vi "_CalcExpress Examples Navigator.vi"   [LabVIEW 2021]
doc: "This VI launches <B>CalcExpress Examples Navigator</B> which will help you to explore CalcExpress examples.\n\nYou can also start the Examples Navigator through <B>Tools>>CalcExpress</B> menu.\n\n::: CalcExpress Toolkit :::\nCopyright (c) 2000-2026 Konstantin Shifershteyn. All rights reserved."
uses:
  vi.lib/addons/CalcExpress/cemisc.llb/[ce] CE component paths - Kind of Path Enum.ctl
panel:
  # "Starting CalcExpress Examples Navigator..."
types:
  T1 = typedef "[ce] CE component paths - Kind of Path Enum.ctl" = enum16{"VIs", "FuncVIs", "Help", "Examples", "Project", "Templates"}
  T2 = enum32{"Invalid", "Standard", "Closed", "Hidden", "Minimized", "Maximized"}
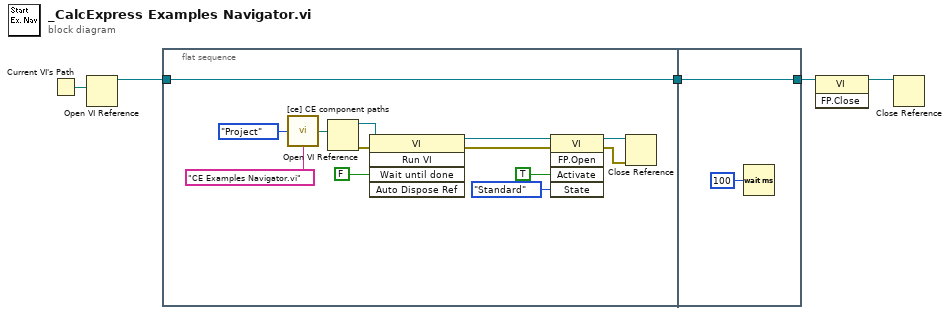
[diagram p0: block diagram]
diagram:
  n1 = Current VI's Path() -> (path=w5:path)
  n2 = Open VI Reference(vi path=w5) -> (vi reference=w2:refnum<vi>)  [unwired: 5 in, 1 out]
  n3 = flat-sequence {
    tunnel: w2 -> [w7]
    tunnel: [w7] -> w1
    tunnel: [w20] -> w4
    tunnel: w1 -> [w20]
    frame #0 {
      n4 = call "[ce] CE component paths.vi"("kind of path"=[ce]_CE_component_paths_-_Kind_of_Path_Enum."Project", "append path"="CE Examples Navigator.vi") -> ("path out"=w15:path)
      n5 = Open VI Reference(vi path=w15) -> (vi reference=w13:refnum<vi>, error out=w12:errorcluster)  [unwired: 5 in]
      n6 = invoke class="VI" method="Run VI"(reference=w13, error in=w12, "Wait until done"=FALSE) -> (reference out=w11:refnum<vi>, error out=w9:errorcluster)  [unwired: 2 in, 3 out]
      n7 = invoke class="VI" method="FP.Open"(reference=w11, error in=w9, "Activate"=TRUE ("Front Panel.Open"), "State"=T2."Standard") -> (reference out=w18:refnum<vi>, error out=w8:errorcluster)  [unwired: 1 in, 3 out]
      n8 = Close Reference(reference=w18, error in (no error)=w8) -> ()  [unwired: 1 out]
    }
    frame #1 {
      n9 = Wait (ms)(milliseconds to wait=u32 100) -> ()  [unwired: 1 out]
    }
  }
  n10 = invoke class="VI" method="FP.Close"(reference=w4) -> (reference out=w3:refnum<vi>)  [unwired: 2 in, 2 out]
  n11 = Close Reference(reference=w3) -> ()  [unwired: 1 in, 1 out]
